vi "Init UI.vi"(8 "error in (no error)":errorcluster, 11 "Sequencing Control in":refnum<class "Sequencing Control.lvclass">) -> (0 "error out":errorcluster, 3 "Sequencing Control out":refnum<class "Sequencing Control.lvclass">)   [LabVIEW 2020, in "VolatusSeqGUI.lvlib" / "Sequencing Control.lvclass"]
uses:
  Sequencing Control.lvclass
  C:/dev/lv20CE/relink/lv-volatus/VolatusGUI/GUI Element/GUI Element.lvclass
  Colors.ctl
  VolatusGUI/GUI Element/GUI Element.lvclass/GUI Element.ctl
  Sequencing Control.lvclass/Sequencing Control.ctl
  VolatusGUI/GUI Element/GUI Element.lvclass
  C:/dev/lv20CE/relink/lv-volatus/VolatusSeqGUI/Sequencing Control/Sequencing Control.lvclass
  C:/dev/lv20CE/relink/lv-volatus/VolatusGUI/OnValueChangeHandler/OnValueChangeHandler.lvclass
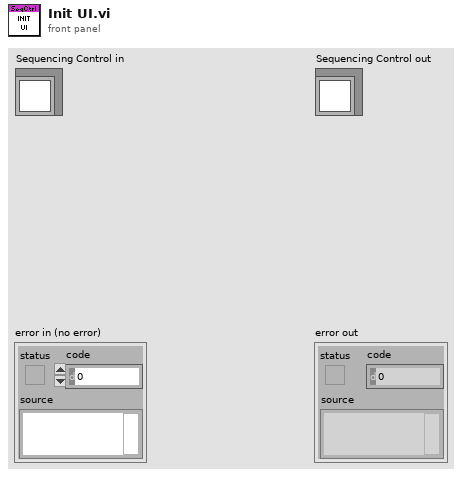
[diagram p1: front panel]
types:
  T1 = typedef "VolatusSeqGUI.lvlib/Sequencing Control.lvclass/Colors.ctl" = cluster{"Default":u32, "Unloaded":u32, "Seq Error":u32, "Loaded Good CRC":u32, "Loaded Bad CRC":u32, "Running Good CRC":u32, "Running Bad CRC":u32}
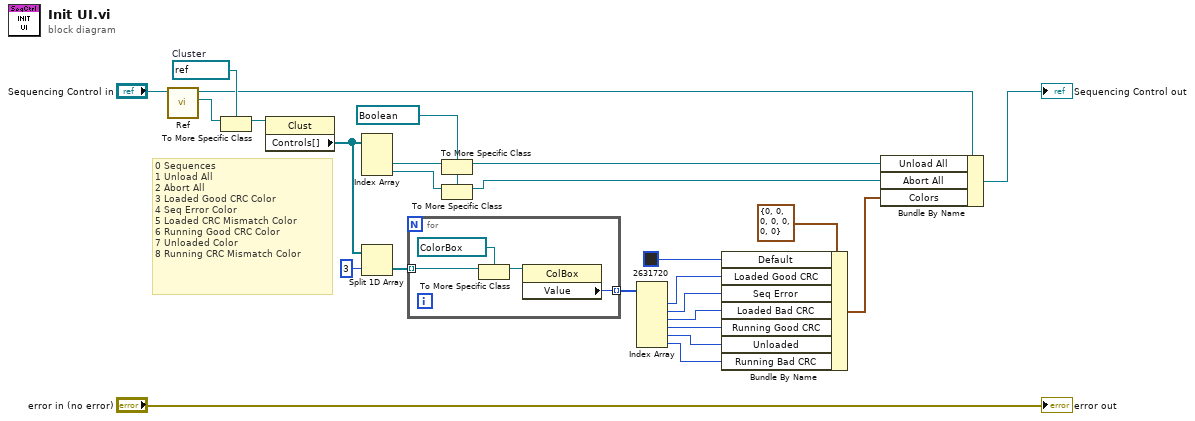
[diagram p0: block diagram]
diagram:
  w20 = refnum<vi> refnum ("Unload All")
  w24 = refnum<vi> refnum  # Cluster
  # "0 Sequences\n1 Unload All\n2 Abort All\n3 Loaded Good CRC Color\n4 Seq Error Color\n5 Loaded CRC Mismatch Color\n6 Running Good CRC Color\n7 Unloaded Color\n8 Running CRC Mismatch Color"
  n1 = call "Ref.vi"("GUI Element in"="Sequencing Control in") -> ("Ref"=w25:refnum<vi>, "GUI Element out"=w13:refnum<class "Sequencing Control.lvclass">)  [unwired: 9 in]
  n2 = To More Specific Class(target class=w24, reference=w25) -> (specific class reference=w23:refnum<vi>)  [unwired: 1 in, 1 out]
  n3 = property class="Clust"(reference=w23) -> ("Controls[]"=w17:refnum<vi>[])  [unwired: 1 in, 2 out]
  n4 = Index Array(array=w17) -> (element #2=w22:refnum<vi>, element #3=w21:refnum<vi>)  [unwired: 3 in, 1 out]
  n5 = Split 1D Array(array=w17, index=3) -> (second subarray=w15:refnum<vi>[])  [unwired: 1 out]
  n6 = for {
    tunnel: w15 -> [w29] mode=indexing
    tunnel: [w26] -> w9 mode=indexing
    n7 = To More Specific Class(target class=refnum<vi> refnum ("Running, CRC Mismatch"), reference=w29) -> (specific class reference=w27:refnum<vi>)  [unwired: 1 in, 1 out]
    n8 = property class="ColBox"(reference=w27) -> ("Value"=w26:u32)  [unwired: 1 in, 2 out]
  }
  n9 = To More Specific Class(target class=w20, reference=w22) -> (specific class reference=w19:refnum<vi>)  [unwired: 1 in, 1 out]
  n10 = To More Specific Class(target class=w20, reference=w21) -> (specific class reference=w18:refnum<vi>)  [unwired: 1 in, 1 out]
  n11 = Index Array(array=w9) -> (element #1=w7:u32, element #2=w6:u32, element #3=w5:u32, element #4=w4:u32, element #5=w3:u32, element #6=w2:u32)  [unwired: 6 in]
  n12 = Bundle By Name(cluster=T1 {"Default"=0, "Unloaded"=0, "Seq Error"=0, "Loaded Good CRC"=0, "Loaded Bad CRC"=0, "Running Good CRC"=0, "Running Bad CRC"=0} ("Colors"), "Default"=u32 2631720, "Loaded Good CRC"=w7, "Seq Error"=w6, "Loaded Bad CRC"=w5, "Running Good CRC"=w4, "Unloaded"=w3, "Running Bad CRC"=w2) -> (w1:T1)
  n13 = Bundle By Name(cluster=w13, "Unload All"=w19, "Abort All"=w18, "Colors"=w1) -> (→"Sequencing Control out":refnum<class "Sequencing Control.lvclass">)
  "error out" <- "error in (no error)"
